vi "macro_PIDController_Execute.vi"() -> ()   [LabVIEW 2019, in "Trajectory_Library.lvlib"]
uses:
  Trajectory_Library.lvlib
panel:
  out "CO-ControlOutput":dbl
  in  "SP-SetPoint":dbl
  in  "PV-Measurement":dbl
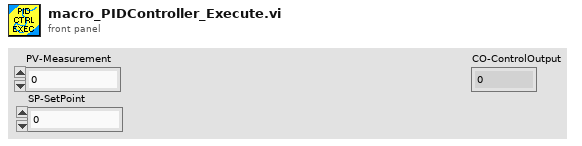
[diagram p1: front panel]
types:
  T1 = typedef "Trajectory_Library.lvlib/PID_TUNING.ctl" = cluster{"Kp":dbl, "Ki":dbl, "Kd":dbl, "MaximumIntegral":dbl, "MinimumIntegral":dbl, "IntegralZone":dbl}
  T2 = typedef "Trajectory_Library.lvlib/PID_INPUT_LIMITS.ctl" = cluster{"MaxInput":dbl, "MinInput":dbl, "Continuous":bool}
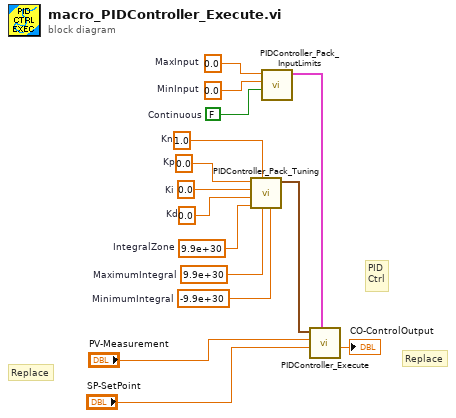
[diagram p0: block diagram]
diagram:
  w1 = 9.9e+30  # IntegralZone
  w5 = 1.0  # Kn
  w6 = 0.0  # MaxInput
  w7 = 0.0  # MinInput
  w8 = FALSE  # Continuous
  w9 = 0.0  # Kp
  w10 = 0.0  # Ki
  w11 = 0.0  # Kd
  w12 = 9.9e+30  # MaximumIntegral
  w13 = -9.9e+30  # MinimumIntegral
  # "Replace"
  # "Replace"
  # "PID\nCtrl"
  n1 = call "PIDController_Pack_Tuning.vi"("MinimumIntegral"=w13, "MaximumIntegral"=w12, "Kn"=w5, "IntegralZone"=w1, "Kd"=w11, "Ki"=w10, "Kp"=w9) -> ("PID Tuning"=w14:T1)  [unwired: 4 in]
  n2 = call "PIDController_Pack_InputLimits.vi"("Continuous"=w8, "MinInput"=w7, "MaxInput"=w6) -> ("PID Input Limits"=w15:T2)  [unwired: 8 in]
  n3 = call "PIDController_Execute.vi"("PID Input Limits"=w15, "SP-SetPoint"="SP-SetPoint", "PV-Measurement"="PV-Measurement", "PID Tuning"=w14) -> ("CO-ControlOutput"=→"CO-ControlOutput":dbl)  [unwired: 5 in, 2 out]
